vi "Construct.vi"(8 "error in (no error)":errorcluster, 9 "App.Args":string[](array[string]), 11 "SolutionBuilder in":refnum<class "SolutionBuilder.lvclass">) -> (0 "error out":errorcluster, 3 "SolutionBuilder out":refnum<class "SolutionBuilder.lvclass">)   [LabVIEW 2019, in "SolutionBuilder.lvlib" / "SolutionBuilder.lvclass"]
uses:
  SolutionBuilder.lvclass
  SolutionBuilder.lvclass/SolutionBuilder.ctl
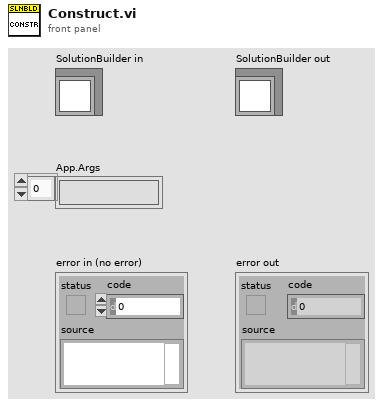
[diagram p1: front panel]
types:
  T1 = typedef "SolutionBuilder.lvlib/SolutionBuilder.lvclass/Options.ctl" = cluster{"Path":path, "Preview?":bool, "Quiet?":bool, "Log file":path, "Success file":path, "Rebuild?":bool, "Keep split projects?":bool, "Version string":string}
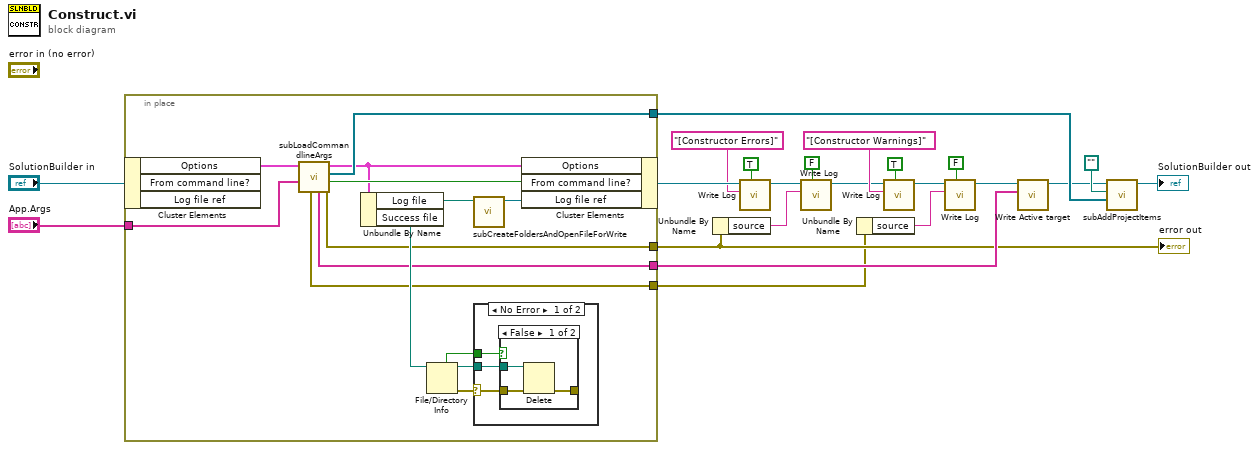
[diagram p0: block diagram]
diagram:
  n1 = in-place {
    in-place-border: [w34] -> w20
    in-place-border: "App.Args" -> [w33]
    in-place-border: [w25] -> w16
    in-place-border: [w24] -> w10
    in-place-border: [w23] -> w2
    n2 = in-place-cluster #1("SolutionBuilder in") -> ("Options"=w36:T1)  [unwired: 2 out]
    n3 = call "subLoadCommandlineArgs.vi"("App.Args"=w33, "Options in"=w36) -> ("error out"=w24:errorcluster, "From command line?"=w35:bool, "Pre-built libraries"=w34:refnum<class "ProjectItem.lvclass">[], "Options"=w32:T1, "Active targets"=w25:string[], "warnings out"=w23:errorcluster)  [unwired: 4 in]
    n4 = Unbundle By Name(w32) -> ("Log file"=w30:path, "Success file"=w29:path)
    n5 = File/Directory Info(path=w29) -> (path out=w27:path, directory=w26:bool, error out=w28:errorcluster)  [unwired: 1 in, 4 out]
    n6 = call "subCreateFoldersAndOpenFileForWrite.vi"("File path"=w30) -> ("File ref"=w31:refnum<file>)  [unwired: 9 in, 1 out]
    n7 = case shown="No Error" w28 {
      selector: w28 -> [w37 _]
      tunnel: w27 -> [w38 _]
      tunnel: w26 -> [w39 _]
      frame No Error {
        n8 = case shown="False" w39 {
          tunnel: w38 -> [w42 _]
          tunnel: w37 -> [w41 _]
          tunnel: [w40 _] -> _
          frame False {
            n9 = Delete(path (use dialog)=w42, error in=w41) -> (error out=w40:errorcluster)  [unwired: 3 in, 2 out]
          }
          frame True {
          }
        }
      }
      frame Error {
      }
    }
    n10 = in-place-cluster #1("Options"=w32, "From command line?"=w35, "Log file ref"=w31) -> (w15:refnum<class "SolutionBuilder.lvclass">)
  }
  "error out" <- w10
  n11 = Unbundle By Name(w10) -> ("source"=w9:string)
  n12 = call "Write Log.vi"("Prepend timestamp"=TRUE, "Log entry"="[Constructor Errors]", "SolutionBuilder in"=w15) -> ("SolutionBuilder out"=w12:refnum<class "SolutionBuilder.lvclass">)  [unwired: 8 in]
  n13 = call "Write Log.vi"("Prepend timestamp"=FALSE, "Log entry"=w9, "SolutionBuilder in"=w12) -> ("SolutionBuilder out"=w3:refnum<class "SolutionBuilder.lvclass">)  [unwired: 8 in]
  n14 = Unbundle By Name(w2) -> ("source"=w8:string)
  n15 = call "Write Log.vi"("Prepend timestamp"=TRUE, "Log entry"="[Constructor Warnings]", "SolutionBuilder in"=w3) -> ("SolutionBuilder out"=w6:refnum<class "SolutionBuilder.lvclass">)  [unwired: 8 in]
  n16 = call "Write Log.vi"("Prepend timestamp"=FALSE, "Log entry"=w8, "SolutionBuilder in"=w6) -> ("SolutionBuilder out"=w1:refnum<class "SolutionBuilder.lvclass">)  [unwired: 8 in]
  n17 = call-dynamic "Write Active target.vi"("Active targets"=w16, "SolutionBuilder in"=w1) -> ("SolutionBuilder out"=w17:refnum<class "SolutionBuilder.lvclass">)  [unwired: 9 in]
  n18 = call "subAddProjectItems.vi"("ProjectItems"=w20, "Owning project"=path "", "SolutionBuilder in"=w17) -> ("SolutionBuilder out"=→"SolutionBuilder out":refnum<class "SolutionBuilder.lvclass">)  [unwired: 7 in, 1 out]
